vi "Record Attributes.vi"(1 "record":T1, 12 "error in":errorcluster) -> (2 "record out":T1, 15 "error out":errorcluster)   [LabVIEW 2026]
doc: "Pass a record with an attribute map through."
uses:
  Record.ctl
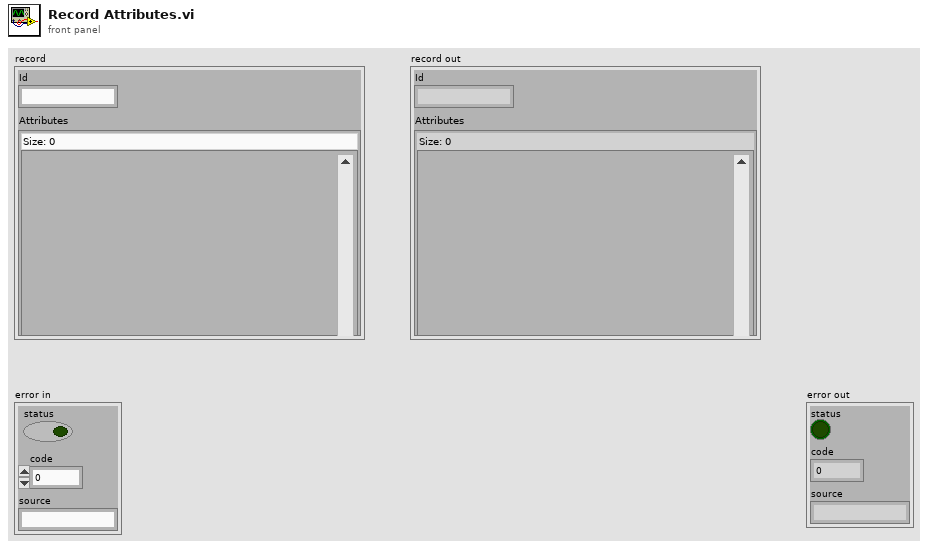
[diagram p1: front panel]
types:
  T1 = typedef "Record.ctl" = cluster{"Id":string, "Attributes":map{string, variant}}
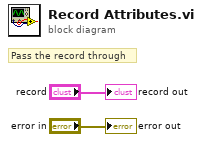
[diagram p0: block diagram]
diagram:
  # "Pass the record through"
  "record out" <- "record"
  "error out" <- "error in"
